vi "Parameters_Build_Stop.vi"(11 "Stop Mode":i32(ring)=11599968 items=["Decelerate"=11599968, "Immediate"=11599969, "Disable Drive"=11599970]) -> (3 "Parameters":dbl[](array[numeric]))   [LabVIEW 2017, in "WordManipulationLibrary.lvlib"]
uses:
  WordManipulationLibrary.lvlib
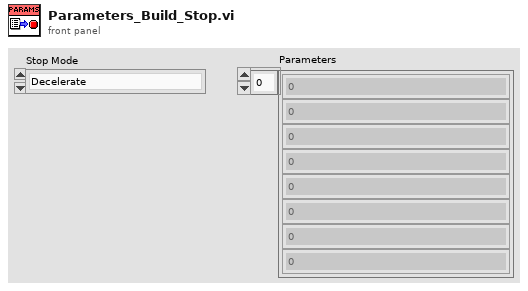
[diagram p1: front panel]
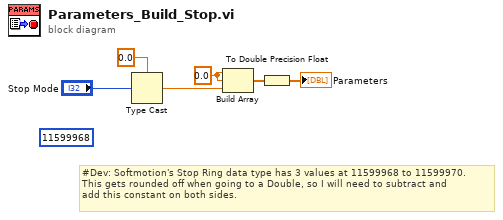
[diagram p0: block diagram]
diagram:
  (unwired) 11599968 ("y")
  w6 = 0.0 ("element")
  # "#Dev: Softmotion's Stop Ring data type has 3 values at 11599968 to 11599970. \nThis gets rounded off when going to a Double, so I will need to subtract and\nadd this constant on both sides."
  n1 = Type Cast(type=0.0 ("element"), x="Stop Mode") -> (*(type *) &x=w2:dbl)
  n2 = Build Array(w6, w6, w2) -> (w4:dbl[])
  n3 = To Double Precision Float(number=w4) -> (double precision float=→"Parameters":dbl[])
